vi "Process.vi"(8 "error in":errorcluster, 11 "Plugin in":refnum<class "Modbus.lvclass">) -> (0 "error out":errorcluster, 3 "Plugin out":refnum<class "Modbus.lvclass">)   [LabVIEW 2026, in "Modbus.lvlib" / "Modbus.lvclass"]
uses:
  Modbus.lvclass
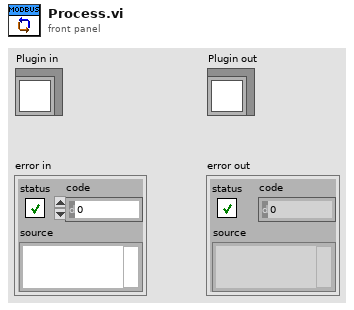
[diagram p1: front panel]
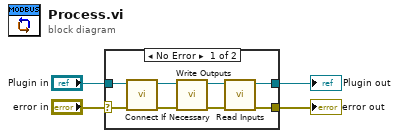
[diagram p0: block diagram]
diagram:
  n1 = case shown="No Error" "error in" {
    selector: "error in" -> [w11 w14]
    tunnel: [w6 w13] -> w2
    tunnel: "Plugin in" -> [w12 w13]
    tunnel: [w5 w14] -> w1
    frame No Error {
      n2 = call "Connect If Necessary.vi"("error in (no error)"=w11, "Plugin in"=w12) -> ("error out"=w10:errorcluster, "Plugin out"=w7:refnum<class "Modbus.lvclass">)  [unwired: 8 in]
      n3 = call "Write Outputs.vi"("error in (no error)"=w10, "Modbus in"=w7) -> ("error out"=w8:errorcluster, "Modbus out"=w9:refnum<class "Modbus.lvclass">)  [unwired: 8 in]
      n4 = call "Read Inputs.vi"("error in (no error)"=w8, "Modbus in"=w9) -> ("error out"=w5:errorcluster, "Modbus out"=w6:refnum<class "Modbus.lvclass">)  [unwired: 8 in]
    }
    frame Error {
    }
  }
  "error out" <- w1
  "Plugin out" <- w2
